vi "Register gRPC Methods.vi"(8 "error in (no error)":errorcluster, 11 "gRPC service in":refnum<class "ThermalChamberController.lvclass">) -> (0 "error out":errorcluster, 3 "gRPC service out":refnum<class "ThermalChamberController.lvclass">)   [LabVIEW 2020, in "thermal-chamber-controller_server.lvlib" / "ThermalChamberController.lvclass"]
uses:
  ThermalChamberController.lvclass
  typeDefs/Server Internal UEs.ctl
  typeDefs/Server Internal Message.ctl
  typeDefs/Server gRPC UEs.ctl
  <vilib>/gRPC/LabVIEW gRPC Library/Server API/typeDefs/gRPCId Cluster.ctl
  <vilib>/gRPC/LabVIEW gRPC Library/Shared/grpcId.ctl
  ThermalChamberController.lvclass/ThermalChamberController.ctl
  <vilib>/gRPC/LabVIEW gRPC Library/grpc-lvsupport-release.lvlib
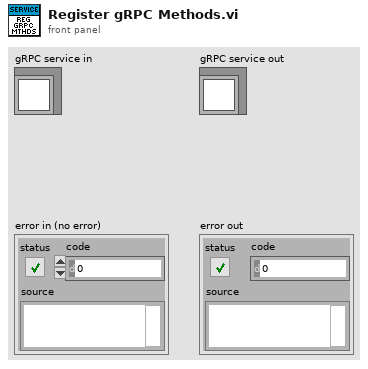
[diagram p1: front panel]
types:
  T1 = typedef "thermal-chamber-controller_server.lvlib/ThermalChamberController.lvclass/Server gRPC UEs.ctl" = cluster{"ThermalChamberController StartModule gRPC UE":refnum<user-event>, "ThermalChamberController ShowModulePanel gRPC UE":refnum<user-event>, "ThermalChamberController HideModulePanel gRPC UE":refnum<user-event>, "ThermalChamberController StopModule gRPC UE":refnum<user-event>, "ThermalChamberController UpdateSetPoint gRPC UE":refnum<user-event>, "ThermalChamberController UpdateRampRate gRPC UE":refnum<user-event>, "ThermalChamberController UpdateHeaterState gRPC UE":refnum<user-event>, "ThermalChamberController SubscribeChamberStatusUpdated gRPC UE":refnum<user-event>, "ThermalChamberController SubscribeSetPointUpdated gRPC UE":refnum<user-event>, "ThermalChamberController SubscribeRampRateUpdated gRPC UE":refnum<user-event>, "ThermalChamberController SubscribeHeaterStateUpdated gRPC UE":refnum<user-event>}
  T2 = typedef "thermal-chamber-controller_server.lvlib/ThermalChamberController.lvclass/Server Internal UEs.ctl" = cluster{"ThermalChamberController StartModule Internal UE":refnum<user-event>, "ThermalChamberController ShowModulePanel Internal UE":refnum<user-event>, "ThermalChamberController HideModulePanel Internal UE":refnum<user-event>, "ThermalChamberController StopModule Internal UE":refnum<user-event>, "ThermalChamberController UpdateSetPoint Internal UE":refnum<user-event>, "ThermalChamberController UpdateRampRate Internal UE":refnum<user-event>, "ThermalChamberController UpdateHeaterState Internal UE":refnum<user-event>, "ThermalChamberController SubscribeChamberStatusUpdated Internal UE":refnum<user-event>, "ThermalChamberController SubscribeSetPointUpdated Internal UE":refnum<user-event>, "ThermalChamberController SubscribeRampRateUpdated Internal UE":refnum<user-event>, "ThermalChamberController SubscribeHeaterStateUpdated Internal UE":refnum<user-event>}
  T3 = typedef "grpc-lvsupport-release.lvlib/grpcId.ctl" = u64
  T4 = typedef "thermal-chamber-controller_server.lvlib/ThermalChamberController.lvclass/Server Internal Message UE.ctl" = refnum<user-event>
  T5 = typedef "grpc-lvsupport-release.lvlib/gRPCId Cluster UE.ctl" = refnum<user-event>
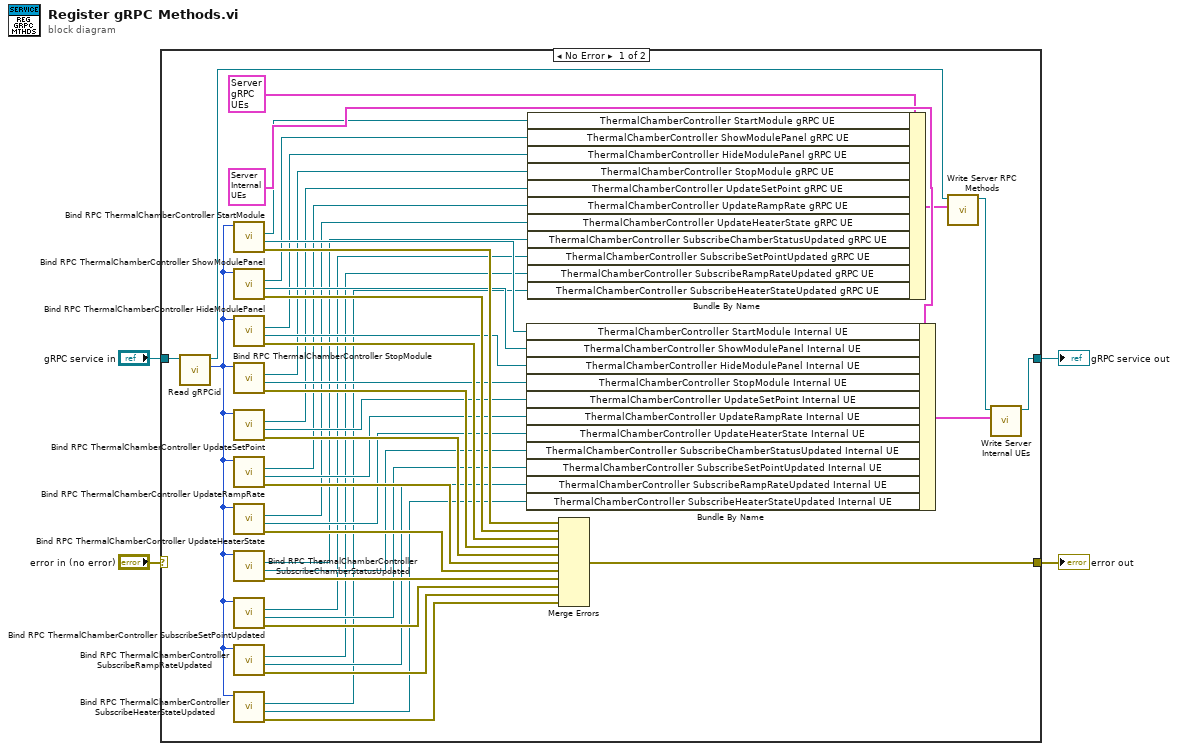
[diagram p0: block diagram]
diagram:
  n1 = case shown="No Error" "error in (no error)" {
    selector: "error in (no error)" -> [_ w48]
    tunnel: "gRPC service in" -> [w39 w49]
    tunnel: [w47 w48] -> w3
    tunnel: [w46 w49] -> w2
    frame No Error {
      n2 = call-dynamic "Read gRPCid.vi"("gRPC service in"=w39) -> ("gRPCid"=w38:T3, "gRPC service out"=w40:refnum<class "ThermalChamberController.lvclass">)  [unwired: 8 in, 1 out]
      n3 = call "Bind RPC ThermalChamberController StartModule.vi"("gRPCid server in"=w38) -> ("error out"=w37:errorcluster, "ThermalChamberController StartModule Internal UE"=w36:T4, "ThermalChamberController StartModule gRPC UE"=w35:T5)  [unwired: 7 in, 1 out]
      n4 = call "Bind RPC ThermalChamberController ShowModulePanel.vi"("gRPCid server in"=w38) -> ("error out"=w34:errorcluster, "ThermalChamberController ShowModulePanel Internal UE"=w32:T4, "ThermalChamberController ShowModulePanel gRPC UE"=w33:T5)  [unwired: 7 in, 1 out]
      n5 = call "Bind RPC ThermalChamberController HideModulePanel.vi"("gRPCid server in"=w38) -> ("error out"=w31:errorcluster, "ThermalChamberController HideModulePanel Internal UE"=w30:T4, "ThermalChamberController HideModulePanel gRPC UE"=w29:T5)  [unwired: 7 in, 1 out]
      n6 = call "Bind RPC ThermalChamberController StopModule.vi"("gRPCid server in"=w38) -> ("error out"=w28:errorcluster, "ThermalChamberController StopModule Internal UE"=w26:T4, "ThermalChamberController StopModule gRPC UE"=w27:T5)  [unwired: 7 in, 1 out]
      n7 = call "Bind RPC ThermalChamberController UpdateSetPoint.vi"("gRPCid server in"=w38) -> ("error out"=w25:errorcluster, "ThermalChamberController UpdateSetPoint Internal UE"=w24:T4, "ThermalChamberController UpdateSetPoint gRPC UE"=w23:T5)  [unwired: 7 in, 1 out]
      n8 = call "Bind RPC ThermalChamberController UpdateRampRate.vi"("gRPCid server in"=w38) -> ("error out"=w22:errorcluster, "ThermalChamberController UpdateRampRate Internal UE"=w20:T4, "ThermalChamberController UpdateRampRate gRPC UE"=w21:T5)  [unwired: 7 in, 1 out]
      n9 = call "Bind RPC ThermalChamberController UpdateHeaterState.vi"("gRPCid server in"=w38) -> ("error out"=w19:errorcluster, "ThermalChamberController UpdateHeaterState Internal UE"=w17:T4, "ThermalChamberController UpdateHeaterState gRPC UE"=w18:T5)  [unwired: 7 in, 1 out]
      n10 = call "Bind RPC ThermalChamberController SubscribeChamberStatusUpdated.vi"("gRPCid server in"=w38) -> ("error out"=w16:errorcluster, "ThermalChamberController SubscribeChamberStatusUpdated Internal UE"=w14:T4, "ThermalChamberController SubscribeChamberStatusUpdated gRPC UE"=w15:T5)  [unwired: 7 in, 1 out]
      n11 = call "Bind RPC ThermalChamberController SubscribeSetPointUpdated.vi"("gRPCid server in"=w38) -> ("error out"=w13:errorcluster, "ThermalChamberController SubscribeSetPointUpdated Internal UE"=w11:T4, "ThermalChamberController SubscribeSetPointUpdated gRPC UE"=w12:T5)  [unwired: 7 in, 1 out]
      n12 = call "Bind RPC ThermalChamberController SubscribeRampRateUpdated.vi"("gRPCid server in"=w38) -> ("error out"=w10:errorcluster, "ThermalChamberController SubscribeRampRateUpdated Internal UE"=w8:T4, "ThermalChamberController SubscribeRampRateUpdated gRPC UE"=w9:T5)  [unwired: 7 in, 1 out]
      n13 = call "Bind RPC ThermalChamberController SubscribeHeaterStateUpdated.vi"("gRPCid server in"=w38) -> ("error out"=w7:errorcluster, "ThermalChamberController SubscribeHeaterStateUpdated Internal UE"=w5:T4, "ThermalChamberController SubscribeHeaterStateUpdated gRPC UE"=w6:T5)  [unwired: 7 in, 1 out]
      n14 = Bundle By Name ("Bundle Internal UEs")(cluster=T2 {"ThermalChamberController StartModule Internal UE"=refnum, "ThermalChamberController ShowModulePanel Internal UE"=refnum, "ThermalChamberController HideModulePanel Internal UE"=refnum, "ThermalChamberController StopModule Internal UE"=refnum, "ThermalChamberController UpdateSetPoint Internal UE"=refnum, "ThermalChamberController UpdateRampRate Internal UE"=refnum, "ThermalChamberController UpdateHeaterState Internal UE"=refnum, "ThermalChamberController SubscribeChamberStatusUpdated Internal UE"=refnum, "ThermalChamberController SubscribeSetPointUpdated Internal UE"=refnum, "ThermalChamberController SubscribeRampRateUpdated Internal UE"=refnum, "ThermalChamberController SubscribeHeaterStateUpdated Internal UE"=refnum} ("Server Internal UEs"), "ThermalChamberController StartModule Internal UE"=w36, "ThermalChamberController ShowModulePanel Internal UE"=w32, "ThermalChamberController HideModulePanel Internal UE"=w30, "ThermalChamberController StopModule Internal UE"=w26, "ThermalChamberController UpdateSetPoint Internal UE"=w24, "ThermalChamberController UpdateRampRate Internal UE"=w20, "ThermalChamberController UpdateHeaterState Internal UE"=w17, "ThermalChamberController SubscribeChamberStatusUpdated Internal UE"=w14, "ThermalChamberController SubscribeSetPointUpdated Internal UE"=w11, "ThermalChamberController SubscribeRampRateUpdated Internal UE"=w8, "ThermalChamberController SubscribeHeaterStateUpdated Internal UE"=w5) -> (w45:T2)
      n15 = Bundle By Name ("Bundle gRPC UEs")(cluster=T1 {"ThermalChamberController StartModule gRPC UE"=refnum, "ThermalChamberController ShowModulePanel gRPC UE"=refnum, "ThermalChamberController HideModulePanel gRPC UE"=refnum, "ThermalChamberController StopModule gRPC UE"=refnum, "ThermalChamberController UpdateSetPoint gRPC UE"=refnum, "ThermalChamberController UpdateRampRate gRPC UE"=refnum, "ThermalChamberController UpdateHeaterState gRPC UE"=refnum, "ThermalChamberController SubscribeChamberStatusUpdated gRPC UE"=refnum, "ThermalChamberController SubscribeSetPointUpdated gRPC UE"=refnum, "ThermalChamberController SubscribeRampRateUpdated gRPC UE"=refnum, "ThermalChamberController SubscribeHeaterStateUpdated gRPC UE"=refnum} ("gRPC Server Method Events"), "ThermalChamberController StartModule gRPC UE"=w35, "ThermalChamberController ShowModulePanel gRPC UE"=w33, "ThermalChamberController HideModulePanel gRPC UE"=w29, "ThermalChamberController StopModule gRPC UE"=w27, "ThermalChamberController UpdateSetPoint gRPC UE"=w23, "ThermalChamberController UpdateRampRate gRPC UE"=w21, "ThermalChamberController UpdateHeaterState gRPC UE"=w18, "ThermalChamberController SubscribeChamberStatusUpdated gRPC UE"=w15, "ThermalChamberController SubscribeSetPointUpdated gRPC UE"=w12, "ThermalChamberController SubscribeRampRateUpdated gRPC UE"=w9, "ThermalChamberController SubscribeHeaterStateUpdated gRPC UE"=w6) -> (w42:T1)
      n16 = Merge Errors(w37, w34, w31, w28, w25, w22, w19, w16, w13, w10, w7) -> (w47:errorcluster)
      n17 = call "Write Server RPC Methods.vi"("Server RPC Methods"=w42, "gRPC service in"=w40) -> ("gRPC service out"=w43:refnum<class "ThermalChamberController.lvclass">)  [unwired: 8 in, 1 out]
      n18 = call "Write Server Internal UEs.vi"("Server Internal UEs"=w45, "gRPC service in"=w43) -> ("gRPC service out"=w46:refnum<class "ThermalChamberController.lvclass">)  [unwired: 8 in, 1 out]
    }
    frame Error {
    }
  }
  "error out" <- w3
  "gRPC service out" <- w2
